vi "Execute.vi"(0 "Session Handle in":T1, 2 "Break at First Step? (F)":bool, 11 "error in (no error)":errorcluster) -> (4 "Session Handle out":T1, 15 "error out":errorcluster)   [LabVIEW 2020, in "TSS.lvlib" / "Execution.lvclass"]
uses:
  Execution.lvclass
  Typedefs/Session Handle.ctl
  Execution.lvclass/Execution.ctl
  Engine/Get Engine Ref.vi
  SequenceFile/Get Ref Prop.vi
  VariableContainer/Get Ref Prop.vi
  VariableContainer/VariableContainer.lvclass
  Engine/Engine.lvclass
  SequenceFile/SequenceFile.lvclass
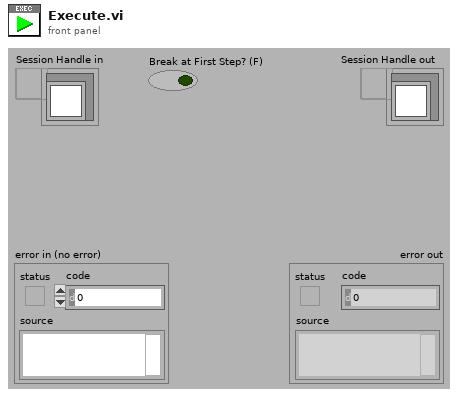
[diagram p1: front panel]
types:
  T1 = typedef "TSS.lvlib/Execution.lvclass/Session Handle.ctl" = refnum<data-value>
  T2 = typedef "TSS.lvlib/SequenceFile.lvclass/Session Handle.ctl" = refnum<data-value>
  T3 = typedef "TSS.lvlib/VariableContainer.lvclass/Session Handle.ctl" = refnum<data-value>
  T4 = typedef "TSS.lvlib/Engine.lvclass/Session Handle.ctl" = refnum<data-value>
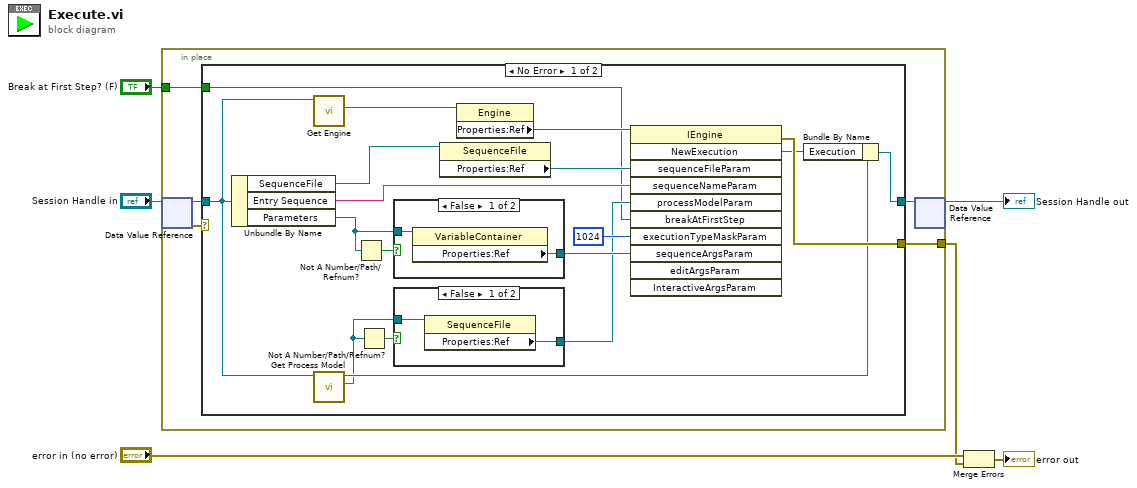
[diagram p0: block diagram]
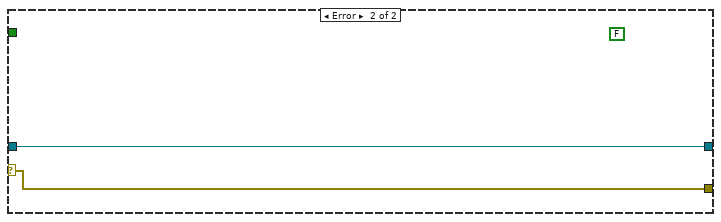
[diagram p4: hidden frame]
diagram:
  n1 = in-place {
    in-place-border: [w8] -> w2
    in-place-border: "Break at First Step? (F)" -> [w7]
    n2 = in-place-dvr #1("Session Handle in") -> (w11:refnum<class "Execution.lvclass">, w9:errorcluster)
    n3 = case shown="No Error" w9 {
      selector: w9 -> [_ w35]
      tunnel: w11 -> [w14 w34]
      tunnel: [w21 w34] -> w10
      tunnel: [w29 w35] -> w8
      tunnel: w7 -> [w12 _]
      frame No Error {
        n4 = Unbundle By Name(w14) -> ("SequenceFile"=w27:T2, "Entry Sequence"=w25:string, "Parameters"=w23:T3)
        n5 = call "Get Engine.vi"("Execution in"=w14) -> ("Engine"=w13:T4)  [unwired: 8 in, 2 out]
        n6 = call "Get Process Model.vi"("Execution in"=w14) -> ("Process Model"=w16:T2, "Execution out"=w18:refnum<class "Execution.lvclass">)  [unwired: 8 in, 1 out]
        n7 = Not A Number/Path/Refnum?(number/path/refnum=w23) -> (NaN/Path/Refnum?=w24:bool)
        n8 = Not A Number/Path/Refnum?(number/path/refnum=w16) -> (NaN/Path/Refnum?=w17:bool)
        n9 = case shown="False" w24 {
          tunnel: w23 -> [w33 _]
          tunnel: [w32 _] -> w22
          frame False {
            n10 = property class="VariableContainer"(reference=w33) -> ("Properties:Ref"=w32:refnum<k7>)  [unwired: 1 in, 2 out]
          }
          frame True {
          }
        }
        n11 = case shown="False" w17 {
          tunnel: w16 -> [w31 _]
          tunnel: [w30 _] -> w15
          frame False {
            n12 = property class="SequenceFile"(reference=w31) -> ("Properties:Ref"=w30:refnum<k7>)  [unwired: 1 in, 2 out]
          }
          frame True {
          }
        }
        n13 = property class="SequenceFile"(reference=w27) -> ("Properties:Ref"=w26:refnum<k7>)  [unwired: 1 in, 2 out]
        n14 = property class="Engine"(reference=w13) -> ("Properties:Ref"=w28:refnum<k7>)  [unwired: 1 in, 2 out]
        n15 = invoke class="IEngine" method="NewExecution"(reference=w28, "sequenceFileParam"=w26, "sequenceNameParam"=w25, "processModelParam"=w15, "breakAtFirstStep"=w12, "executionTypeMaskParam"=1024, "sequenceArgsParam"=w22) -> (error out=w29:errorcluster, "NewExecution"=w19:refnum<k7>)  [unwired: 4 in, 9 out]
        n16 = Bundle By Name(cluster=w18, "Execution"=w19) -> (w21:refnum<class "Execution.lvclass">)
      }
      frame Error {
        (unwired) FALSE ("Auto Release")
      }
    }
    n17 = in-place-dvr #1(w10) -> (→"Session Handle out":T1)  [unwired: 1 out]
  }
  n18 = Merge Errors("error in (no error)", w2) -> (→"error out":errorcluster)
